vi "DAQ Switch.vi"(8 "Error In":errorcluster caption="错误输入", 9 "Command In":string, 10 "Time and Data In":T1, 11 "Sample Settings":T2={"设备信息"={"初始索引子集"=[], "模拟信号采集通道"="Dev1", "数字-供电"="", "数字-光控"="", "光控设备"="", "光电设备分离？"=FALSE, "光谱保存路径"=path "", "环数"=0}, "测量控制"={"测头拿起"=FALSE, "起始保存"=FALSE, "测头供电"=TRUE, "测头出光"=TRUE}, "测量"={"每波长测量次数"=5, "波长"=[0, 0, 0, 0, 0, 0], "起始周期"=0, "起始测量周期"=0}, "等待"={"等待时间(s)"=0.0, "等待方式"=FALSE, "每x周期/点等待"=8, "等待时"=enum."无电无光"}, "校准"={"暗电流校准值初值"=[], "温度校准值"=[0.0, 0.0, 0.0, 0.0, 0.0, 0.0, 0.00013, 0.00013, 0.00013, 0.00013, 0.00013, 0.00013], "校准模式"=enum."逐周期"}, "图表相关"={"文件-时间"=""}, "CSM"={"CSM Name"=""}}) -> (0 "Error Out":errorcluster caption="错误输出", 1 "Command Out":string, 2 "Off时刻":timestamp)   [LabVIEW 2026, in "UI-无创.lvlib" / "Acquisition.lvlib"]
uses:
  Acquisition.lvlib
  Supports/Sample Settings.ctl
  Supports/Time and Data_OP.ctl
  <vilib>/DAQmx/write.llb/DAQmx Write (Digital U32 1Chan 1Samp).vi
  <vilib>/DAQmx/miscellaneous.llb/DAQmx Fill In Error Info.vi
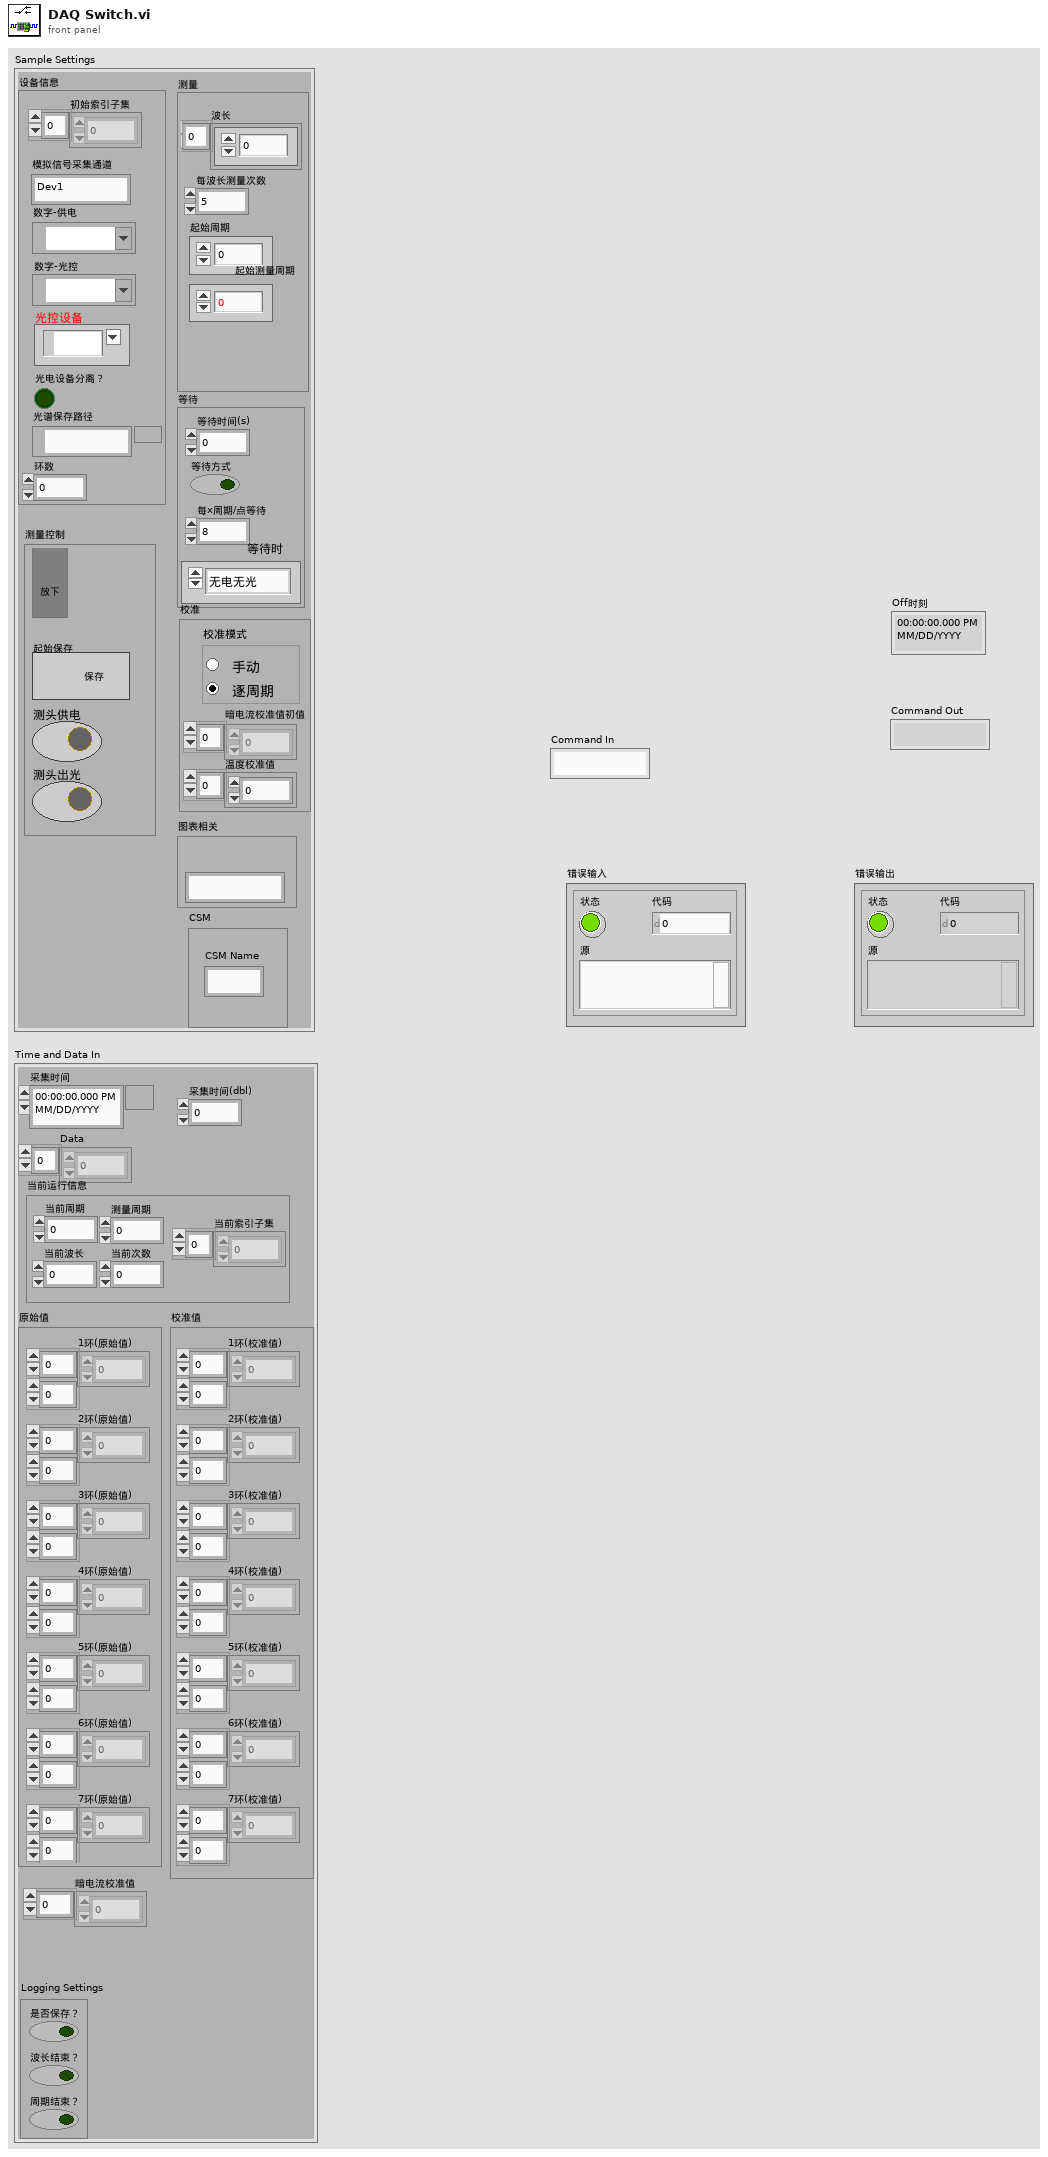
[diagram p1: front panel]
types:
  T1 = typedef "UI-无创.lvlib/Time and Data_OP.ctl" = cluster{"采集时间":timestamp, "采集时间(dbl)":dbl, "Data":dbl[], "当前运行信息":cluster{"当前周期":i32, "当前次数":i32, "测量周期":i32, "当前索引子集":i8[], "当前波长":i32}, "暗电流校准值":dbl[], "Logging Settings":cluster{"是否保存？":bool, "波长结束？":bool, "周期结束？":bool}, "原始值":cluster{"1环(原始值)":dbl[][], "2环(原始值)":dbl[][], "3环(原始值)":dbl[][], "4环(原始值)":dbl[][], "5环(原始值)":dbl[][], "6环(原始值)":dbl[][], "7环(原始值)":dbl[][]}, "校准值":cluster{"1环(校准值)":dbl[][], "2环(校准值)":dbl[][], "3环(校准值)":dbl[][], "4环(校准值)":dbl[][], "5环(校准值)":dbl[][], "6环(校准值)":dbl[][], "7环(校准值)":dbl[][]}}
  T2 = typedef "UI-无创.lvlib/Sample Settings.ctl" = cluster{"设备信息":cluster{"初始索引子集":i8[], "模拟信号采集通道":string, "数字-供电":refnum<k21>, "数字-光控":refnum<k21>, "光控设备":tag, "光电设备分离？":bool, "光谱保存路径":path, "环数":u8}, "测量控制":cluster{"测头拿起":bool, "起始保存":bool, "测头供电":bool, "测头出光":bool}, "测量":cluster{"每波长测量次数":i32, "波长":i32[], "起始周期":i32, "起始测量周期":i32}, "等待":cluster{"等待时间(s)":dbl, "等待方式":bool, "每x周期/点等待":i32, "等待时":enum16{"无电无光", "有电无光", "无电有光", "有电有光"}}, "校准":cluster{"暗电流校准值初值":dbl[], "温度校准值":dbl[], "校准模式":T3}, "图表相关":cluster{"文件-时间":string}, "CSM":cluster{"CSM Name":string}}
  T3 = typedef "UI-无创.lvlib/暗电流校准模式.ctl" = enum32{"手动", "逐周期"}
  T4 = cluster{"Sample Settings":T2, "Time and Data In":T1}
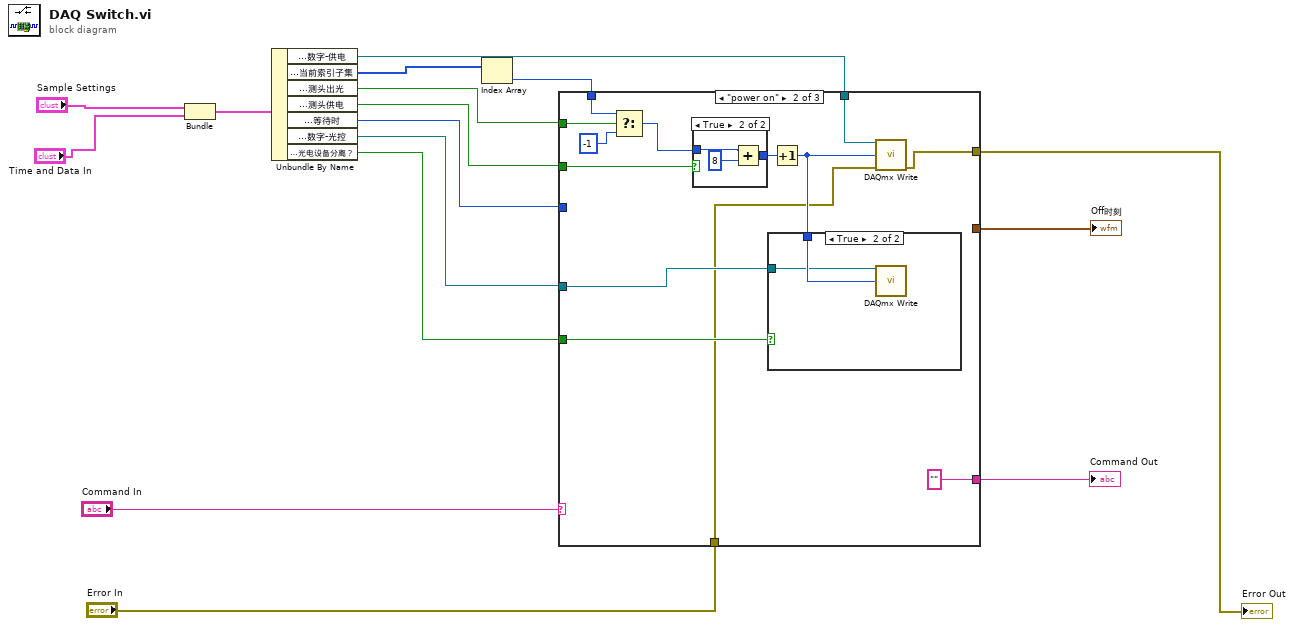
[diagram p0: block diagram]
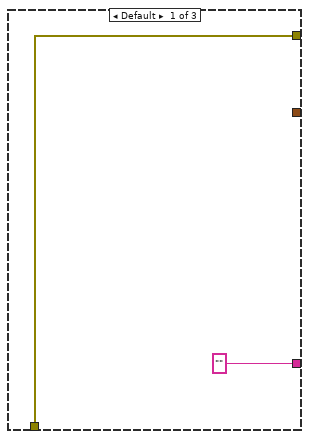
[diagram p2: hidden frame]
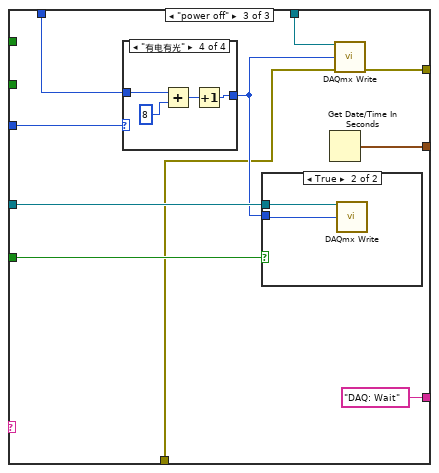
[diagram p5: hidden frame]
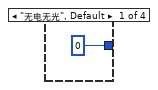
[diagram p7: hidden frame]
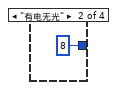
[diagram p8: hidden frame]
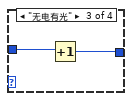
[diagram p9: hidden frame]
diagram:
  n1 = Bundle("Sample Settings"="Sample Settings", "Time and Data In"="Time and Data In") -> (w3:T4)  [unwired: 1 in]
  n2 = Unbundle By Name(w3) -> ("Sample Settings.设备信息.数字-供电"=w14:refnum<k21>, "Time and Data In.当前运行信息.当前索引子集"=w15:i8[], "Sample Settings.测量控制.测头出光"=w8:bool, "Sample Settings.测量控制.测头供电"=w7:bool, "Sample Settings.等待.等待时"=w11:enum16{"无电无光", "有电无光", "无电有光", "有电有光"}, "Sample Settings.设备信息.数字-光控"=w13:refnum<k21>, "Sample Settings.设备信息.光电设备分离？"=w12:bool)
  n3 = Index Array(array=w15) -> (element=w16:i8)  [unwired: 1 in]
  n4 = case shown="\"power on\"" "Command In" {
    tunnel: w16 -> [_ w25 w45]
    tunnel: w7 -> [_ w30 _]
    tunnel: [_ _ w47] -> w6
    tunnel: w14 -> [_ w29 w46]
    tunnel: w11 -> [_ _ w44]
    tunnel: w13 -> [_ w27 w43]
    tunnel: w12 -> [_ w26 w42]
    tunnel: w8 -> [_ w24 _]
    tunnel: ["" "" "DAQ: Wait"] -> w9
    tunnel: [w17 w21 w39] -> w5
    tunnel: "Error In" -> [w17 w20 w38]
    frame Default {
    }
    frame "power on" {
      n5 = Select(t=w25, s=w24, f=-1) -> (s? t:f=w23:i32)
      n6 = case shown="True" w30 {
        tunnel: w23 -> [w34 w37]
        tunnel: [w34 w35] -> w31
        frame False {
        }
        frame True {
          n7 = Add(x=w37, y=8) -> (x+y=w35:i32)
        }
      }
      n8 = Increment(x=w31) -> (x+1=w28:i32)
      n9 = case shown="True" w26 {
        tunnel: w28 -> [_ w33]
        tunnel: w27 -> [_ w32]
        frame False {
        }
        frame True {
          n10 = call-poly <vilib>:"DAQmx Write.vi"("task/channels in"=w32, "data"=w33) -> ()  [unwired: 11 in, 3 out]
        }
      }
      n11 = call-poly <vilib>:"DAQmx Write.vi"("task/channels in"=w29, "data"=w28, "error in"=w20) -> ("error out"=w21:errorcluster)  [unwired: 10 in, 2 out]
    }
    frame "power off" {
      n12 = case shown="\"有电有光\"" w44 {
        tunnel: w45 -> [_ _ w53 w56]
        tunnel: [0 8 w52 w54] -> w41
        frame "无电无光", Default {
        }
        frame "有电无光" {
        }
        frame "无电有光" {
          n13 = Increment(x=w53) -> (x+1=w52:i8)
        }
        frame "有电有光" {
          n14 = Add(x=w56, y=8) -> (x+y=w55:i32)
          n15 = Increment(x=w55) -> (x+1=w54:i32)
        }
      }
      n16 = case shown="True" w42 {
        tunnel: w43 -> [_ w49]
        tunnel: w41 -> [_ w48]
        frame False {
        }
        frame True {
          n17 = call-poly <vilib>:"DAQmx Write.vi"("task/channels in"=w49, "data"=w48) -> ()  [unwired: 11 in, 3 out]
        }
      }
      n18 = Get Date/Time In Seconds() -> (seconds since 1Jan1904=w47:timestamp)
      n19 = call-poly <vilib>:"DAQmx Write.vi"("task/channels in"=w46, "data"=w41, "error in"=w38) -> ("error out"=w39:errorcluster)  [unwired: 10 in, 2 out]
    }
  }
  "Command Out" <- w9
  "Off时刻" <- w6
  "Error Out" <- w5
